vi "ce exmpl - compare 1D arrays.vi"(5 "checking array B":dbl[](array[numeric]) format="%.2f", 6 "standard array A":dbl[](array[numeric]) format="%.2f") -> (0 "arrays are different":bool, 1 "array sizes are not equal":bool, 2 "max relative difference":T1={"index"=-1, "absolute difference"=0.0, "relative difference, %"=0.0} {"relative difference, %" format="%#.6g"; "absolute difference" format="%#.6g"}, 3 "max absolute difference":T1={"index"=-1, "absolute difference"=0.0, "relative difference, %"=0.0} {"relative difference, %" format="%#.6g"; "absolute difference" format="%#.6g"})   [LabVIEW 2021]
doc: "::: CalcExpress Toolkit :::\nCopyright (c) 2000-2026 Konstantin Shifershteyn. All rights reserved."
uses:
  ce exmpl - 1D difference info.ctl
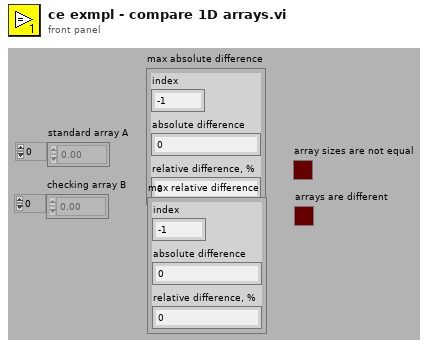
[diagram p1: front panel]
types:
  T1 = typedef "ce exmpl - 1D difference info.ctl" = cluster{"index":i32, "absolute difference":dbl, "relative difference, %":dbl}
  T2 = cluster{"index":i32, "absolute deviation":dbl, "relative deviation %":dbl}
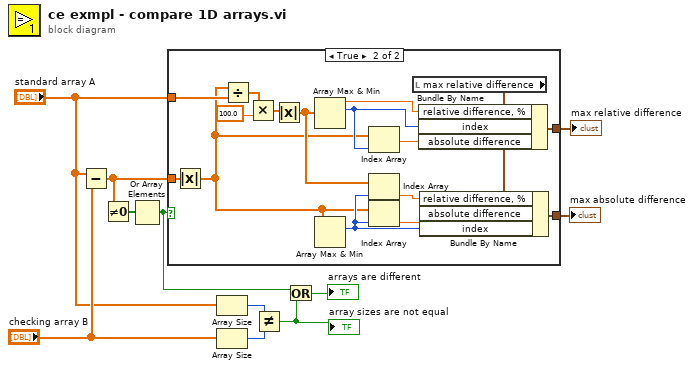
[diagram p0: block diagram]
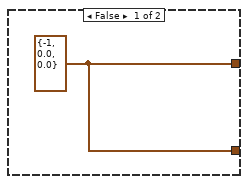
[diagram p2: hidden frame]
diagram:
  n1 = Subtract(x="standard array A", y="checking array B") -> (x-y=w3:dbl[])
  n2 = Not Equal To 0?(x=w3) -> (x != 0?=w2:bool[])
  n3 = Or Array Elements(Boolean array=w2) -> (logical OR=w1:bool)
  n4 = case shown="True" w1 {
    tunnel: "standard array A" -> [_ w22]
    tunnel: [w12 w19] -> w7
    tunnel: [w12 w16] -> w5
    tunnel: w3 -> [_ w14]
    frame False {
      w12 = T2 {"index"=-1, "absolute deviation"=0.0, "relative deviation %"=0.0} ("max relative deviation")
    }
    frame True {
      n5 = Absolute Value(x=w14) -> (abs(x)=w13:dbl[])
      n6 = Divide(x=w13, y=w22) -> (x/y=w27:dbl[])
      n7 = Multiply(x=w27, y=100.0) -> (x*y=w28:dbl[])
      n8 = Absolute Value(x=w28) -> (abs(x)=w21:dbl[])
      n9 = Array Max & Min(array=w21) -> (max value=w15:dbl, max index (indices)=w25:i32)  [unwired: 2 out]
      n10 = Array Max & Min(array=w13) -> (max index (indices)=w23:i32)  [unwired: 3 out]
      n11 = Index Array(array=w13, index=w25) -> (element=w24:dbl)
      n12 = Index Array(array=w21, index=w23) -> (element=w18:dbl)
      n13 = Index Array(array=w13, index=w23) -> (element=w17:dbl)
      n14 = local read "max relative difference"() -> (w20:T1)
      n15 = Bundle By Name(cluster=w20, "relative difference, %"=w15, "index"=w25, "absolute difference"=w24) -> (w16:T1)
      n16 = Bundle By Name(cluster=w20, "relative difference, %"=w18, "absolute difference"=w17, "index"=w23) -> (w19:T1)
    }
  }
  "max absolute difference" <- w7
  "max relative difference" <- w5
  n17 = Array Size(array="standard array A") -> (size(s)=w11:i32)
  n18 = Array Size(array="checking array B") -> (size(s)=w10:i32)
  n19 = Not Equal?(x=w11, y=w10) -> (x != y?=w6:bool)
  "array sizes are not equal" <- w6
  n20 = Or(x=w1, y=w6) -> (x .or. y?=→"arrays are different":bool)
